vi "Test App Removing Process Triggers Broadcast.vi"(8 "error in (no error)":errorcluster, 11 "Rig Test in":refnum<class "Application Dev Test.lvclass">) -> (0 "error out":errorcluster, 3 "Rig Test out":refnum<class "Application Dev Test.lvclass">)   [LabVIEW 2020, in "Application Dev Test.lvclass"]
uses:
  Application Dev Test.lvclass
  C:/Program Files (x86)/National Instruments/LabVIEW 2020/vi.lib/Astemes/LUnit/Test Case.lvclass
  source/Framework/Process/Process.lvclass
  C:/git/astemes-triarc-framework/source/Framework/Logging/Logging.lvclass
  source/Framework/Process/Process.lvclass/Process.ctl
  source/Framework/Application/Application.lvclass/Application.ctl
  source/Framework/Synchronous Request Callback/Synchronous Request Callback.lvclass/Synchronous Request Callback.ctl
  <vilib>/Astemes/LUnit/Test Case.lvclass/Test Case.ctl
  9bca6f49-129a-4f19-9b67-4f930979b2f3.vi
  source/Framework/Process/Public/Lifecycle/Get Lifecycle State.vi
  source/Framework/Application/Private/Add Process to Map.vi
  source/Framework/Application/Private/Throw Error If Process Already in App.vi
  source/Framework/Process/Protected/Messaging/Send Message.vi
  source/Framework/Process/Protected/SubVIs/Set Context.vi
  source/Framework/Application/Private/Remove Process from App.vi
  source/Framework/Application/Private/Parse Process Name.vi
  source/Framework/Application/Private/Remove Process from Map.vi
  source/Framework/Process/Protected/SubVIs/Clear Context.vi
  source/Framework/Broadcast Event Helpers/Execution timer.vi
  <vilib>/Astemes/LUnit/Append Pass Result.vi
  <vilib>/Astemes/LUnit/Append Fail Result.vi
  <vilib>/Astemes/LUnit/Describe Comparison.vi
  <vilib>/Astemes/LUnit/Compare Variants.vi
  source/Framework/Process/Private/SubVIs/Wait for finish.vi
  source/Framework/Process/Private/SubVIs/Set Lifecycle State.vi
  <vilib>/Utility/error.llb/Clear Errors.vi
  source/Framework/Application/Public/Get Process.vi
  source/Framework/Process/Private/SubVIs/Handle Debug Data.vi
  source/Framework/Process/Protected/Messaging/Request Message.vi
  <vilib>/AdvancedString/Delimited String to 1D String Array.vi
  <vilib>/Astemes/LUnit/Variant to string.vi
  source/Framework/Application/Private/Retrieve Process from App.vi
  source/Framework/Application/Private/Get Process from Map.vi
  source/Framework/Logging/Log Debug.vi
  <vilib>/AdvancedString/1D String Array to Delimited String.vi
  <vilib>/Utility/High Resolution Relative Seconds.vi
  source/Framework/Synchronous Request Callback/Create.vi
  source/Framework/Process/Protected/Messaging/Async Request Message.vi
  source/Framework/Application/Application.lvclass
  C:/git/astemes-triarc-framework/source/Framework/Process/Process.lvclass
  source/Framework/Synchronous Request Callback/Synchronous Request Callback.lvclass
  C:/git/astemes-triarc-framework/source/Framework/Callback/Callback.lvclass
  <vilib>/Utility/error.llb/Error Cluster From Error Code.vi
  source/Framework/Process/Private/SubVIs/Wait for Response Message.vi
  source/Framework/Broadcast Event Dequeuers/Dequeue Broadcast Message.vi
  <vilib>/Utility/Data Type/Get Type Information.vi
  <vilib>/Utility/LVClass/Get LV Class Name.vi
  source/Framework/Callback/Callback.lvclass
  source/Framework/Logging/Logging.lvclass
  Application Dev Test.lvclass/Application Dev Test.ctl
  source/Framework/Broadcast Event Dequeuers/Broadcast Event Dequeuers.lvlib
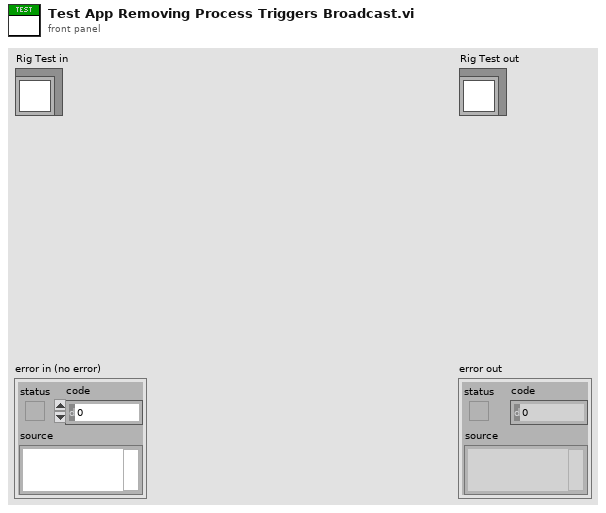
[diagram p1: front panel]
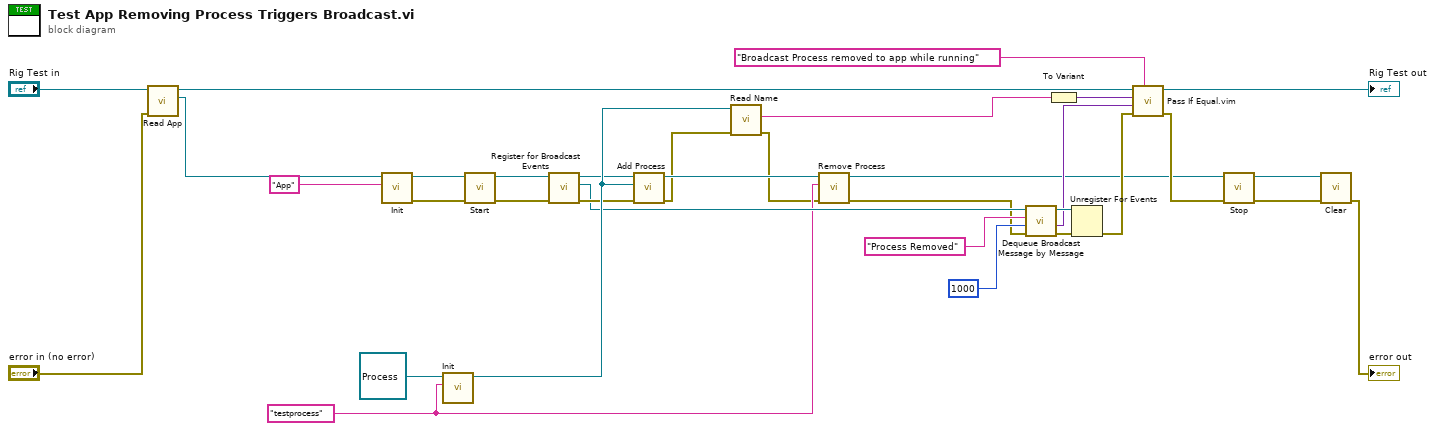
[diagram p0: block diagram]
diagram:
  w4 = "testprocess" ("Name")
  n1 = call "Read App.vi"("error in (no error)"="error in (no error)", "Application Test In"="Rig Test in") -> ("App out"=w33:refnum<class "Application.lvclass">, "Application Test Out"=w24:refnum<class "Application Dev Test.lvclass">)  [unwired: 7 in, 1 out]
  n2 = call-dynamic "Init.vi"("Name"="App", "Process In"=w33) -> ("error out"=w25:errorcluster, "Process Out"=w26:refnum<class "Application.lvclass">)  [unwired: 8 in]
  n3 = call-dynamic "Init.vi"("Name"=w4, "Process In"=refnum<class "Process.lvclass"> refnum ("Process.lvclass")) -> ("Process Out"=w23:refnum<class "Process.lvclass">)  [unwired: 8 in, 1 out]
  n4 = call "Start.vi"("error in (no error)"=w25, "Process In"=w26) -> ("error out"=w27:errorcluster, "Process Out"=w17:refnum<class "Application.lvclass">)  [unwired: 7 in, 1 out]
  n5 = call "Register for Broadcast Events.vi"("error in (no error)"=w27, "Process In"=w17) -> ("error out"=w18:errorcluster, "Event Registration Refnum Out"=w14:refnum<event-registration>, "Process Out"=w16:refnum<class "Application.lvclass">)  [unwired: 7 in]
  n6 = call "Add Process.vi"("error in (no error)"=w18, "Process"=w23, "Application In"=w16) -> ("error out"=w2:errorcluster, "Application Out"=w6:refnum<class "Application.lvclass">)  [unwired: 7 in]
  n7 = call "Read Name.vi"("error in (no error)"=w2, "Process In"=w23) -> ("error out"=w3:errorcluster, "Qualified Name"=w15:string)  [unwired: 6 in, 2 out]
  n8 = call "Remove Process.vi"("error in (no error)"=w3, "Process Name"=w4, "Application In"=w6) -> ("error out"=w1:errorcluster, "Application Out"=w5:refnum<class "Application.lvclass">)  [unwired: 6 in, 1 out]
  n9 = call "Dequeue Broadcast Message by Message.vi"("error in (no error)"=w1, "Timeout (-1)"=1000, "Message"="Process Removed", "Event Registration Refnum"=w14) -> ("error out"=w13:errorcluster, "Message Data"=w10:variant, "Event Registration Refnum Out"=w11:refnum<event-registration>)  [unwired: 3 in, 2 out]
  n10 = To Variant(anything=w15) -> (Variant=w7:variant)
  n11 = Unregister For Events(event registration refnum=w11, error in=w13) -> (error out=w12:errorcluster)
  n12 = call "Pass If Equal.vim"("Description"="Broadcast Process removed to app while running", "error in (no error)"=w12, "Actual"=w10, "Expected"=w7, "LUnit Test Case In"=w24) -> ("error out"=w29:errorcluster, "LUnit Test Case Out"=→"Rig Test out":refnum<class "Application Dev Test.lvclass">)  [unwired: 5 in]
  n13 = call "Stop.vi"("error in (no error)"=w29, "Process In"=w5) -> ("error out"=w21:errorcluster, "Process Out"=w20:refnum<class "Application.lvclass">)  [unwired: 7 in, 1 out]
  n14 = call-dynamic "Clear.vi"("error in (no error)"=w21, "Application In"=w20) -> ("error out"=→"error out":errorcluster)  [unwired: 9 in]
